vi "Gear pusher.vi"(3 "Extend":bool=TRUE, 4 "Cylinder_Devref":T1={"DevStatus"={"status"=FALSE, "code"=0, "source"=""}, "Pneumatics Control Module"=0, "Forward Solenoid Channel"=enum."Invalid", "Reverse Solenoid Channel"=enum."Invalid"}) -> ()   [LabVIEW 2016]
uses:
  <vilib>/Rock Robotics/WPI/Solenoid/WPI_SolenoidDevRef.ctl
  <vilib>/Rock Robotics/WPI/Solenoid/WPI_SolenoidChannel.ctl
  <vilib>/Rock Robotics/WPI/Solenoid/WPI_SolenoidValue.ctl
  Global_Var-RefNum/Global_Var_Other.vi
  <vilib>/Rock Robotics/WPI/Solenoid/WPI_SolenoidSetEnum.vi
  ArgosLib/ArgosLib.lvlib
panel:
  in  "Manual_Place":bool
  in  "TravelTime (ms)":u32=1000
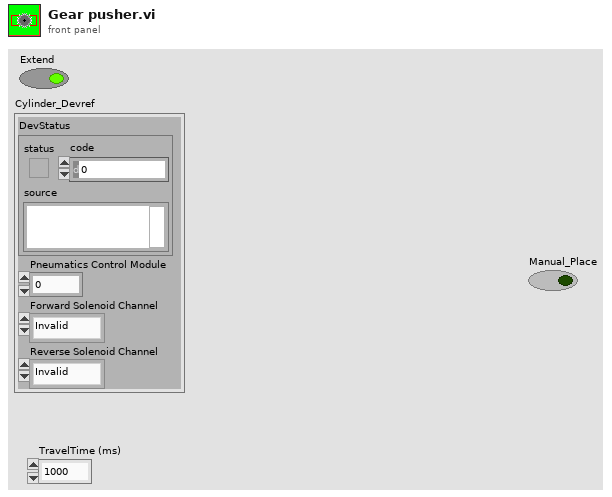
[diagram p1: front panel]
types:
  T1 = typedef "WPI_SolenoidDevRef.ctl" = cluster{"DevStatus":errorcluster, "Pneumatics Control Module":u8, "Forward Solenoid Channel":T2, "Reverse Solenoid Channel":T2}
  T2 = typedef "WPI_SolenoidChannel.ctl" = enum8{"Solenoid 0", "Solenoid 1", "Solenoid 2", "Solenoid 3", "Solenoid 4", "Solenoid 5", "Solenoid 6", "Solenoid 7", "Invalid"}
  T3 = typedef "WPI_SolenoidValue.ctl" = enum16{"Off", "On", "Forward", "Reverse"}
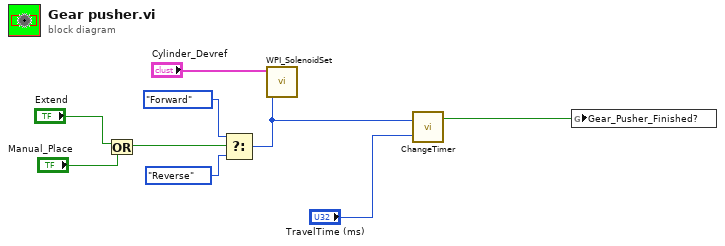
[diagram p0: block diagram]
diagram:
  n1 = Or(x="Extend", y="Manual_Place") -> (x .or. y?=w2:bool)
  n2 = Select(t=WPI_SolenoidValue."Forward" ("Value"), s=w2, f=WPI_SolenoidValue."Reverse" ("Value")) -> (s? t:f=w6:T3)
  n3 = call-poly <vilib>:"WPI_SolenoidSet.vi"("Value"=w6, "SolenoidDevRef"="Cylinder_Devref") -> ()  [unwired: 8 in, 2 out]
  n4 = call "ChangeTimer.vi"("TravelTime (ms)"="TravelTime (ms)", "CheckValue"=w6) -> ("Finished?"=w5:bool)  [unwired: 1 in]
  n5 = global write "Global_Var_Other.vi" "Gear_Pusher_Finished?"(w5) -> ()
